vi "Creation entete fichier.vi"(1 "Commentaire":string) -> (0 "Entête fichier":string)   [LabVIEW 2022 SP3]
uses:
  Variables globales/Variable glob Leybold.vi
  Variables globales/Variable glob Edwards.vi
  Variables globales/Variable glob Keller.vi
  Variables globales/Variable glob Pt.vi
  Variables globales/Variable glob Th.vi
  Variables globales/Variables glob EUROTHERM.vi
  Variables globales/Variable globale compteurs.vi
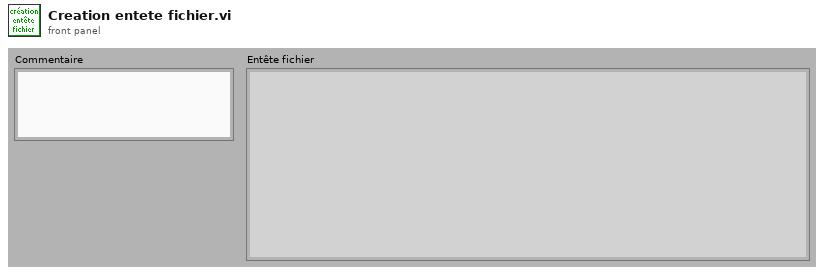
[diagram p1: front panel]
types:
  T1 = cluster{"Nom tache compteurs":refnum<k21>, "Noms des compteurs":string[], "Selection":bool[], "Init compteurs":dbl[], "Noms compteurs selectionnes":string[]}
  T2 = cluster{"Noms voies select acqui 1COM":string[]}[]
  T3 = cluster{"Nom tache Pt":refnum<k21>, "Noms des Pt":string[], "Nb Pt":i16, "Selection Pt":bool[], "Nom Pt selectionnees":string[]}[]
  T4 = cluster{"Nom tache Th":refnum<k21>, "Noms des Th":string[], "Nb Th":i16, "Selection Th":bool[], "Nom Th selectionnes":string[]}[]
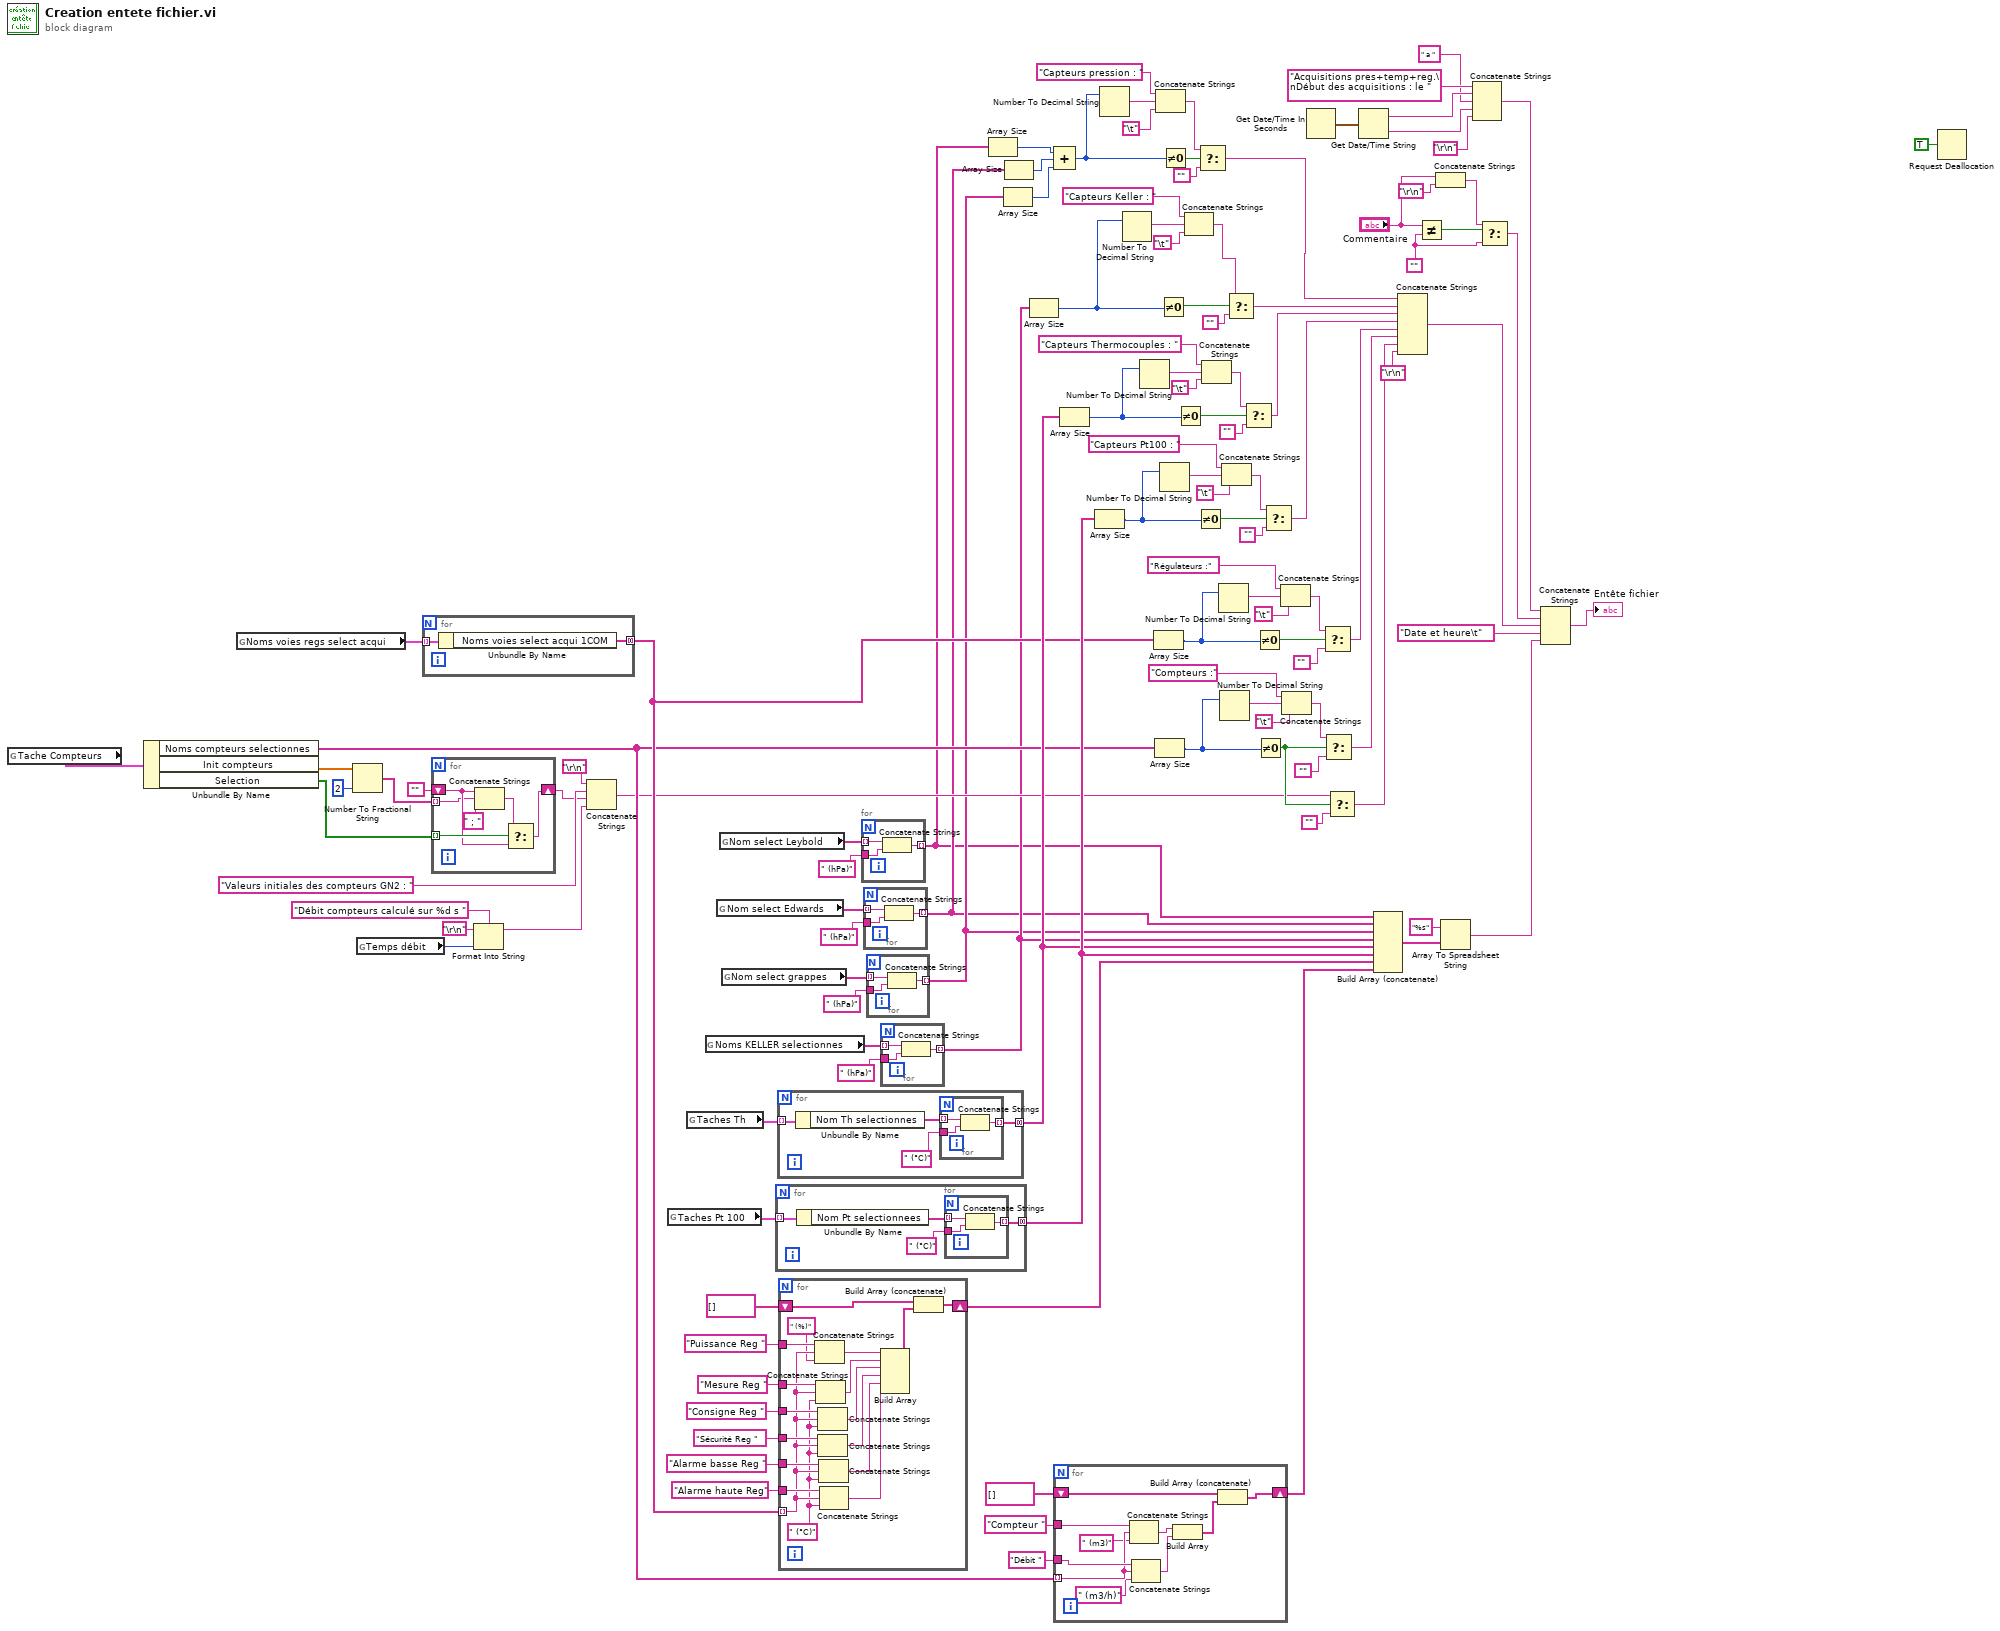
[diagram p0: block diagram]
diagram:
  w15 = ""
  n1 = global read "Variable globale compteurs.vi" "Tache Compteurs"() -> (w55:T1)
  n2 = Unbundle By Name(w55) -> ("Noms compteurs selectionnes"=w45:string[], "Init compteurs"=w30:dbl[], "Selection"=w29:bool[])
  n3 = global read "Variables glob EUROTHERM.vi" "Noms voies regs select acqui"() -> (w57:T2)
  n4 = Number To Fractional String(number=w30, precision (6)=i16 2 ("précision (6)")) -> (F-format string=w28:string[])  [unwired: 2 in]
  n5 = global read "Variable globale compteurs.vi" "Temps débit"() -> (w43:u16)
  n6 = for {
    tunnel: w57 -> [w121] mode=indexing
    tunnel: [w120] -> w56 mode=concatenating
    n7 = Unbundle By Name(w121) -> ("Noms voies select acqui 1COM"=w120:string[])
  }
  n8 = for {
    tunnel: w29 -> [w127] mode=indexing
    tunnel: w28 -> [w124] mode=indexing
    shift-right: [w126] -> w26
    shift-left: "" -> [w125]
    n9 = Concatenate Strings(w125, w124, " ; " ("séparateur (Tabulation)")) -> (w123:string)
    n10 = Select(t=w123, s=w127, f=w125) -> (s? t:f=w126:string)
  }
  n11 = Format Into String(format string="Débit compteurs calculé sur %d s ", initial string="\r\n", w43) -> (resulting string=w35:string)  [unwired: 1 in, 1 out]
  n12 = Concatenate Strings("\r\n", "Valeurs initiales des compteurs GN2 : ", w26, w35) -> (w34:string)
  n13 = global read "Variable glob Pt.vi" "Taches Pt 100"() -> (w69:T3)
  n14 = global read "Variable glob Th.vi" "Taches Th"() -> (w67:T4)
  n15 = global read "Variable glob Keller.vi" "Noms KELLER selectionnes"() -> (w10:string[])
  n16 = global read "Variable glob Edwards.vi" "Nom select Edwards"() -> (w4:string[])
  n17 = global read "Variable glob Leybold.vi" "Nom select Leybold"() -> (w2:string[])
  n18 = global read "Variable glob Edwards.vi" "Nom select grappes"() -> (w7:string[])
  n19 = for {
    tunnel: w69 -> [w131] mode=indexing
    tunnel: [w128] -> w68 mode=concatenating
    n20 = Unbundle By Name(w131) -> ("Nom Pt selectionnees"=w130:string[])
    n21 = for {
      tunnel: w130 -> [w134] mode=indexing
      tunnel: " (°C)" -> [w133]
      tunnel: [w132] -> w128 mode=indexing
      n22 = Concatenate Strings(w134, w133) -> (w132:string)
    }
  }
  n23 = for {
    tunnel: w67 -> [w138] mode=indexing
    tunnel: [w135] -> w66 mode=concatenating
    n24 = Unbundle By Name(w138) -> ("Nom Th selectionnes"=w136:string[])
    n25 = for {
      tunnel: w136 -> [w141] mode=indexing
      tunnel: " (°C)" -> [w140]
      tunnel: [w139] -> w135 mode=indexing
      n26 = Concatenate Strings(w141, w140) -> (w139:string)
    }
  }
  n27 = for {
    tunnel: w56 -> [w153] mode=indexing
    tunnel: "Puissance Reg " -> [w159]
    tunnel: "Mesure Reg " -> [w158]
    tunnel: "Consigne Reg " -> [w157]
    tunnel: "Sécurité Reg " -> [w156]
    tunnel: "Alarme basse Reg " -> [w155]
    tunnel: "Alarme haute Reg" -> [w154]
    shift-right: [w144] -> w58
    shift-left: string[] [] -> [w145]
    w142 = " (°C)"
    n28 = Concatenate Strings(w159, w153, " (%)") -> (w152:string)
    n29 = Concatenate Strings(w158, w153, w142) -> (w151:string)
    n30 = Concatenate Strings(w157, w153, w142) -> (w150:string)
    n31 = Concatenate Strings(w156, w153, w142) -> (w149:string)
    n32 = Concatenate Strings(w155, w153, w142) -> (w148:string)
    n33 = Concatenate Strings(w154, w153, w142) -> (w147:string)
    n34 = Build Array(w152, w151, w150, w149, w148, w147) -> (w146:string[])
    n35 = Build Array (concatenate)(w145, w146) -> (w144:string[])
  }
  n36 = for {
    tunnel: w2 -> [w162] mode=indexing
    tunnel: " (hPa)" -> [w161]
    tunnel: [w160] -> w1 mode=indexing
    n37 = Concatenate Strings(w162, w161) -> (w160:string)
  }
  n38 = for {
    tunnel: w4 -> [w165] mode=indexing
    tunnel: " (hPa)" -> [w164]
    tunnel: [w163] -> w3 mode=indexing
    n39 = Concatenate Strings(w165, w164) -> (w163:string)
  }
  n40 = for {
    tunnel: w7 -> [w168] mode=indexing
    tunnel: " (hPa)" -> [w167]
    tunnel: [w166] -> w6 mode=indexing
    n41 = Concatenate Strings(w168, w167) -> (w166:string)
  }
  n42 = for {
    tunnel: w10 -> [w171] mode=indexing
    tunnel: " (hPa)" -> [w170]
    tunnel: [w169] -> w9 mode=indexing
    n43 = Concatenate Strings(w171, w170) -> (w169:string)
  }
  n44 = Array Size(array=w1) -> (size(s)=w114:i32)
  n45 = Array Size(array=w6) -> (size(s)=w75:i32)
  n46 = Array Size(array=w3) -> (size(s)=w113:i32)
  n47 = Array Size(array=w9) -> (size(s)=w104:i32)
  n48 = Compound Arithmetic op=ADD(w114, w113, w75) -> (w110:i32)
  n49 = for {
    tunnel: w45 -> [w176] mode=indexing
    tunnel: "Compteur " -> [w181]
    shift-right: [w178] -> w44
    shift-left: string[] [] -> [w180]
    tunnel: "Débit " -> [w177]
    n50 = Concatenate Strings(w181, w176, " (m3)") -> (w175:string)
    n51 = Concatenate Strings(w177, w176, " (m3/h)") -> (w174:string)
    n52 = Build Array(w175, w174) -> (w179:string[])
    n53 = Build Array (concatenate)(w180, w179) -> (w178:string[])
  }
  n54 = Array Size(array=w66) -> (size(s)=w95:i32)
  n55 = Array Size(array=w68) -> (size(s)=w89:i32)
  n56 = Number To Decimal String(number=w110) -> (decimal integer string=w108:string)  [unwired: 1 in]
  n57 = Number To Decimal String(number=w104) -> (decimal integer string=w105:string)  [unwired: 1 in]
  n58 = Number To Decimal String(number=w95) -> (decimal integer string=w98:string)  [unwired: 1 in]
  n59 = Array Size(array=w56) -> (size(s)=w83:i32)
  n60 = Array Size(array=w45) -> (size(s)=w47:i32)
  n61 = Concatenate Strings("Capteurs pression : ", w108, "\t") -> (w107:string)
  n62 = Not Equal To 0?(x=w104) -> (x != 0?=w103:bool)
  n63 = Number To Decimal String(number=w89) -> (decimal integer string=w94:string)  [unwired: 1 in]
  n64 = Not Equal To 0?(x=w110) -> (x != 0?=w112:bool)
  n65 = Not Equal To 0?(x=w95) -> (x != 0?=w99:bool)
  n66 = Concatenate Strings("Capteurs Keller : ", w105, "\t") -> (w102:string)
  n67 = Not Equal To 0?(x=w89) -> (x != 0?=w93:bool)
  n68 = Select(t=w107, s=w112, f="") -> (s? t:f=w88:string)
  n69 = Concatenate Strings("Capteurs Thermocouples : ", w98, "\t") -> (w100:string)
  n70 = Number To Decimal String(number=w83) -> (decimal integer string=w78:string)  [unwired: 1 in]
  n71 = Number To Decimal String(number=w47) -> (decimal integer string=w50:string)  [unwired: 1 in]
  n72 = Concatenate Strings("Capteurs Pt100 : ", w94, "\t") -> (w92:string)
  n73 = Select(t=w102, s=w103, f="") -> (s? t:f=w87:string)
  n74 = Select(t=w100, s=w99, f="") -> (s? t:f=w85:string)
  n75 = Not Equal To 0?(x=w83) -> (x != 0?=w79:bool)
  n76 = Not Equal To 0?(x=w47) -> (x != 0?=w40:bool)
  n77 = Select(t=w92, s=w93, f="") -> (s? t:f=w86:string)
  n78 = Concatenate Strings("Régulateurs :", w78, "\t") -> (w80:string)
  n79 = Concatenate Strings("Compteurs :", w50, "\t") -> (w49:string)
  n80 = Get Date/Time In Seconds() -> (seconds since 1Jan1904=w39:timestamp)
  n81 = Select(t=w80, s=w79, f="") -> (s? t:f=w77:string)
  n82 = Select(t=w49, s=w40, f="") -> (s? t:f=w46:string)
  n83 = Select(t=w34, s=w40, f="") -> (s? t:f=w33:string)
  n84 = Get Date/Time String(seconds (now)=w39) -> (date string=w24:string, time string=w22:string)  [unwired: 2 in]
  n85 = Build Array (concatenate)(w1, w3, w6, w9, w66, w68, w58, w44) -> (w115:string[])
  n86 = Concatenate Strings(w88, w87, w85, w86, w77, w46, w33, "\r\n") -> (w84:string)
  n87 = Not Equal?(x="Commentaire", y=w15) -> (x != y?=w20:bool)
  n88 = Concatenate Strings("Commentaire", "\r\n") -> (w16:string)
  n89 = Array To Spreadsheet String(array=w115, 3:"%s" ("chaîne de format")) -> (spreadsheet string=w118:string)  [unwired: 1 in]
  n90 = Concatenate Strings("Acquisitions pres+temp+reg.\nDébut des acquisitions : le ", w24, " a ", w22, "\r\n") -> (w13:string)
  n91 = Select(t=w16, s=w20, f=w15) -> (s? t:f=w14:string)
  n92 = Concatenate Strings(w13, w14, w84, "Date et heure\t", w118) -> (→"Entête fichier":string)
  n93 = Request Deallocation(TRUE ("flag")) -> ()
